vi "Battery Health Checker.vi"(11 "error in":errorcluster) -> (15 "error out":errorcluster)   [LabVIEW 2026]
doc: "Top-level UI of the AA battery health checker. Opens the NI-DMM named in DMM Resource and polls Read Battery Voltage every 200 ms. A battery is detected when |V| >= 0.20 V on 3 consecutive polls; then Measure Battery and Classify Battery run once, the result is shown and a row (time, chemistry, charge, OCV, internal resistance, description) is appended to History. After |V| < 0.10 V on 3 consecutive polls the result is cleared and the VI waits for the next battery. Stop or an error ends the loop; the DMM session is then closed and error out carries the error of the run and of the close."
panel:
  in  "Stop":bool
  out "History":string[][](table)
  out "Measurement":T1
  out "Description":string
  out "Charge (%)":dbl
  out "Chemistry":T2(ring)
  out "Status":string
  out "Battery Present":bool
  out "Live Voltage (V)":dbl
  in  "DMM Resource":refnum<k15>="PXI1Slot3"
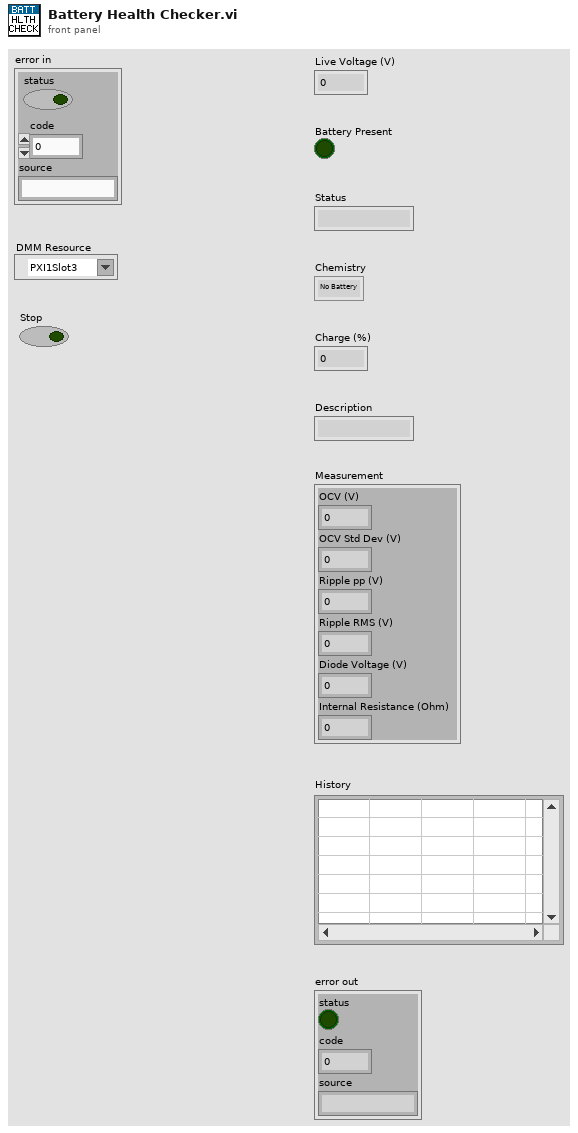
[diagram p1: front panel]
types:
  T1 = cluster{"OCV (V)":dbl, "OCV Std Dev (V)":dbl, "Ripple pp (V)":dbl, "Ripple RMS (V)":dbl, "Diode Voltage (V)":dbl, "Internal Resistance (Ohm)":dbl}
  T2 = enum16{"No Battery", "Reversed Polarity", "Alkaline", "Ni-MH", "Alkaline or Ni-MH", "Li-ion 1.5V (BMS)", "Depleted", "Unknown"}
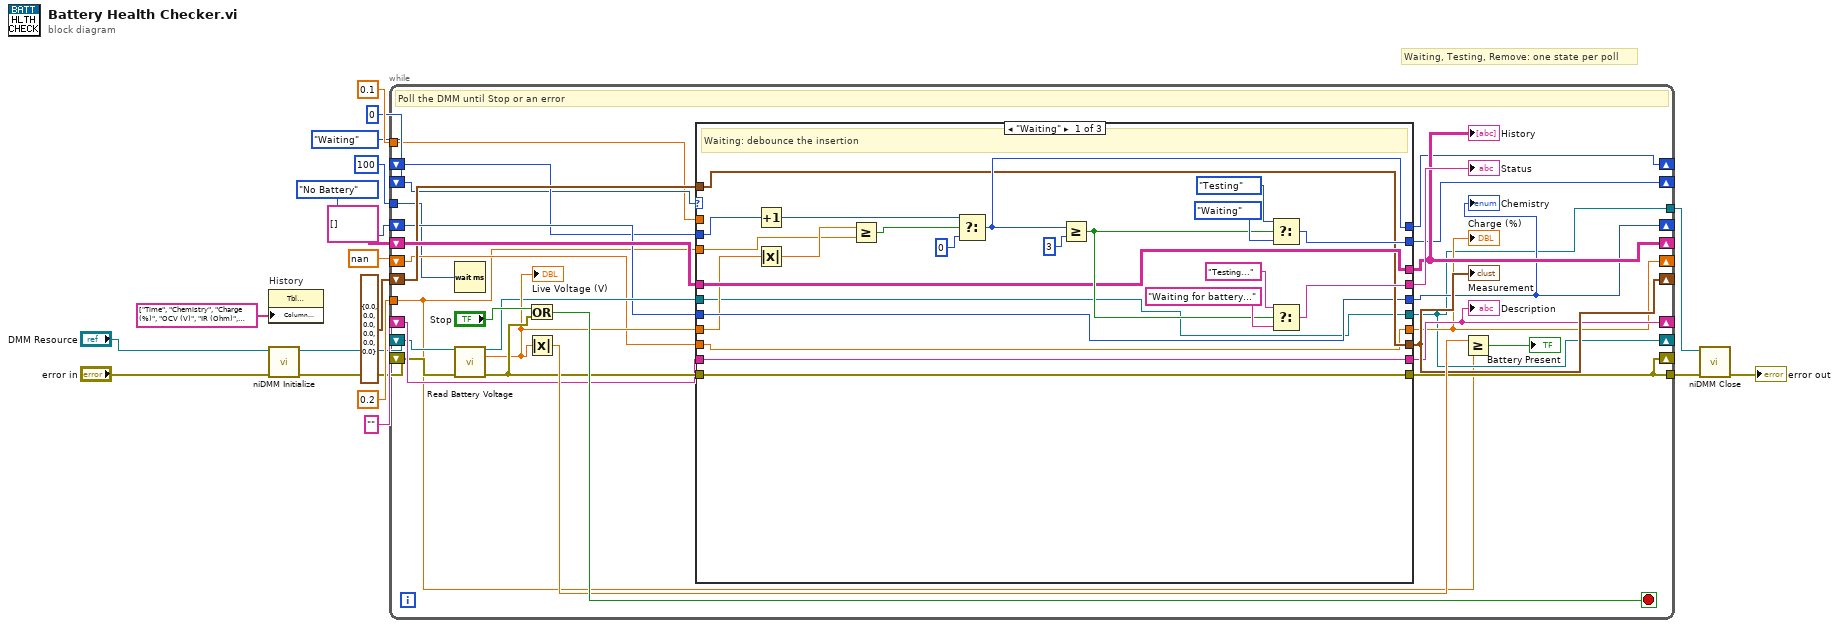
[diagram p0: block diagram]
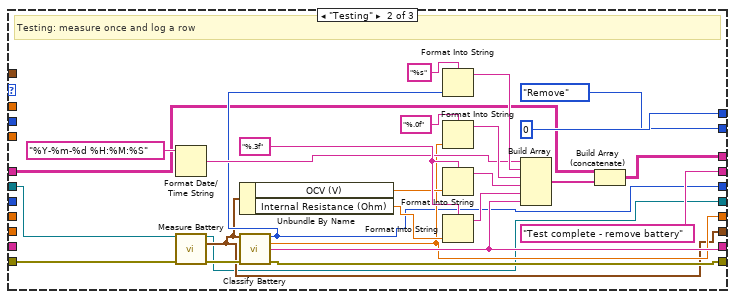
[diagram p2: hidden frame]
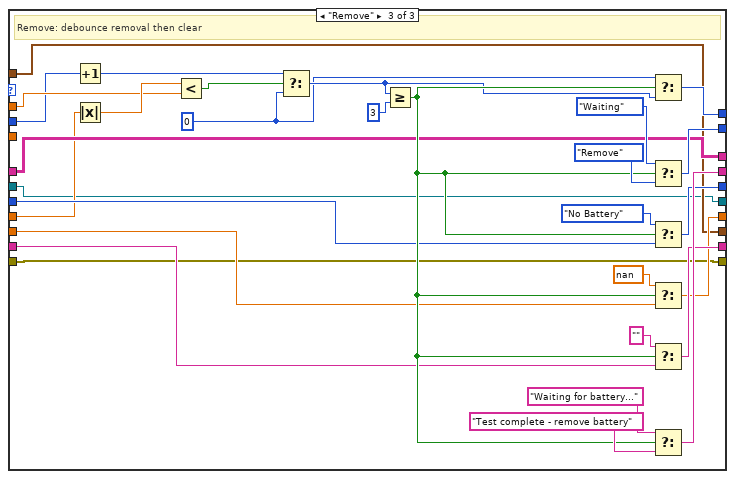
[diagram p3: hidden frame]
diagram:
  # "Waiting, Testing, Remove: one state per poll"
  n1 = property on="History" class="Tbl (strict)"("Column Header Strings[]"=string[] ["Time", "Chemistry", "Charge (%)", "OCV (V)", "IR (Ohm)", "Description"]) -> ()  [unwired: 2 in, 2 out]
  n2 = call <instrlib>:"niDMM Initialize.vi"("error in (no error)"="error in", "Instrument Descriptor"="DMM Resource") -> ("error out"=w4:errorcluster, "instrument handle out"=w5:refnum<k15>)  [unwired: 8 in]
  n3 = while {
    tunnel: 100 ("milliseconds to wait") -> [w19]
    tunnel: 0.2 ("present threshold") -> [w20]
    tunnel: 0.1 ("removed threshold") -> [w21]
    shift-right: [w27] -> _
    shift-left: enum16{"Waiting", "Testing", "Remove"}."Waiting" ("initial state") -> [w26]
    shift-right: [w29] -> _
    shift-left: 0 ("initial count") -> [w28]
    shift-right: [w31] -> _
    shift-left: T2."No Battery" ("initial Chemistry") -> [w30]
    shift-right: [w33] -> _
    shift-left: nan ("initial Charge") -> [w32]
    shift-right: [w35] -> _
    shift-left: "" ("initial Description") -> [w34]
    shift-right: [w37] -> _
    shift-left: T1 {"OCV (V)"=0.0, "OCV Std Dev (V)"=0.0, "Ripple pp (V)"=0.0, "Ripple RMS (V)"=0.0, "Diode Voltage (V)"=0.0, "Internal Resistance (Ohm)"=0.0} ("initial Measurement") -> [w36]
    shift-right: [w39] -> _
    shift-left: string[][] [] ("initial History") -> [w38]
    shift-right: [w23] -> _
    shift-left: w5 -> [w22]
    shift-right: [w25] -> _
    shift-left: w4 -> [w24]
    tunnel: [w23] -> w16
    tunnel: [w25] -> w17
    stop <- w47 stop-if-true
    # "Poll the DMM until Stop or an error"
    n4 = Wait (ms)(milliseconds to wait=w19) -> ()  [unwired: 1 out]
    n5 = call "Read Battery Voltage.vi"("instrument handle"=w22, "error in"=w24) -> ("instrument handle out"=w40:refnum<k15>, "Voltage (V)"=w41:dbl, "error out"=w42:errorcluster)  [unwired: 11 in]
    "Live Voltage (V)" <- w41
    n6 = Or(x="Stop", y=w42) -> (x .or. y?=w47:bool)
    n7 = Absolute Value(x=w41) -> (abs(x)=w43:dbl)
    n8 = case shown="\"Waiting\"" w26 {
      tunnel: w28 -> [w50 _ w99]
      tunnel: w20 -> [w52 _ _]
      tunnel: w30 -> [w53 _ w101]
      tunnel: w32 -> [w54 _ w102]
      tunnel: w34 -> [w55 _ w103]
      tunnel: w36 -> [w56 _ w104]
      tunnel: w38 -> [w57 w73 w105]
      tunnel: w21 -> [_ _ w106]
      tunnel: [w53 w77 w119] -> w31
      tunnel: [w54 w78 w121] -> w33
      tunnel: [w55 w79 w123] -> w35
      tunnel: [w56 w75 w104] -> w37
      tunnel: [w57 w93 w105] -> w39
      tunnel: w40 -> [w48 w71 w97]
      tunnel: w42 -> [w49 w72 w98]
      tunnel: w41 -> [w51 _ w100]
      tunnel: [w48 w74 w97] -> w23
      tunnel: [w49 w80 w98] -> w25
      tunnel: [w62 0 ("count") w114] -> w29
      tunnel: [w67 enum16{"Waiting", "Testing", "Remove"}."Remove" ("next state") w117] -> w27
      tunnel: [w70 "Test complete - remove battery" ("Status") w126] -> w45
      frame "Waiting" {
        # "Waiting: debounce the insertion"
        n9 = Increment(x=w50) -> (x+1=w60:i32)
        n10 = Absolute Value(x=w51) -> (abs(x)=w58:dbl)
        n11 = Greater Or Equal?(x=w58, y=w52) -> (x >= y?=w59:bool)
        n12 = Select(t=w60, s=w59, f=0) -> (s? t:f=w62:i32)
        n13 = Greater Or Equal?(x=w62, y=3) -> (x >= y?=w64:bool)
        n14 = Select(t=enum16{"Waiting", "Testing", "Remove"}."Testing", s=w64, f=enum16{"Waiting", "Testing", "Remove"}."Waiting") -> (s? t:f=w67:enum16{"Waiting", "Testing", "Remove"})
        n15 = Select(t="Testing...", s=w64, f="Waiting for battery...") -> (s? t:f=w70:string)
      }
      frame "Testing" {
        w89 = "%.3f" ("format string")
        # "Testing: measure once and log a row"
        n16 = Format Date/Time String(time format string (%c)="%Y-%m-%d %H:%M:%S") -> (date/time string=w82:string)  [unwired: 1 in, 1 out]
        n17 = call "Measure Battery.vi"("instrument handle"=w71, "error in"=w72) -> ("instrument handle out"=w74:refnum<k15>, "Measurement"=w75:T1, "error out"=w76:errorcluster)  [unwired: 11 in]
        n18 = Unbundle By Name(w75) -> ("OCV (V)"=w87:dbl, "Internal Resistance (Ohm)"=w88:dbl)
        n19 = call "Classify Battery.vi"("Measurement"=w75, "error in"=w76) -> ("Chemistry"=w77:T2, "Charge (%)"=w78:dbl, "Description"=w79:string, "error out"=w80:errorcluster)  [unwired: 10 in]
        n20 = Format Into String(format string="%s", w77) -> (resulting string=w84:string)  [unwired: 2 in, 1 out]
        n21 = Format Into String(format string="%.0f", w78) -> (resulting string=w86:string)  [unwired: 2 in, 1 out]
        n22 = Format Into String(format string=w89, w87) -> (resulting string=w90:string)  [unwired: 2 in, 1 out]
        n23 = Format Into String(format string=w89, w88) -> (resulting string=w91:string)  [unwired: 2 in, 1 out]
        n24 = Build Array(w82, w84, w86, w90, w91, w79) -> (w92:string[])
        n25 = Build Array (concatenate)(w73, w92) -> (w93:string[][])
      }
      frame "Remove" {
        w110 = 0 ("f")
        # "Remove: debounce removal then clear"
        n26 = Increment(x=w99) -> (x+1=w109:i32)
        n27 = Absolute Value(x=w100) -> (abs(x)=w107:dbl)
        n28 = Less?(x=w107, y=w106) -> (x < y?=w108:bool)
        n29 = Select(t=w109, s=w108, f=w110) -> (s? t:f=w111:i32)
        n30 = Greater Or Equal?(x=w111, y=3) -> (x >= y?=w113:bool)
        n31 = Select(t=w110, s=w113, f=w111) -> (s? t:f=w114:i32)
        n32 = Select(t=enum16{"Waiting", "Testing", "Remove"}."Waiting", s=w113, f=enum16{"Waiting", "Testing", "Remove"}."Remove") -> (s? t:f=w117:enum16{"Waiting", "Testing", "Remove"})
        n33 = Select(t=T2."No Battery", s=w113, f=w101) -> (s? t:f=w119:T2)
        n34 = Select(t=nan, s=w113, f=w102) -> (s? t:f=w121:dbl)
        n35 = Select(t="", s=w113, f=w103) -> (s? t:f=w123:string)
        n36 = Select(t="Waiting for battery...", s=w113, f="Test complete - remove battery") -> (s? t:f=w126:string)
      }
    }
    "Status" <- w45
    "Chemistry" <- w31
    "Charge (%)" <- w33
    "Description" <- w35
    "Measurement" <- w37
    "History" <- w39
    n37 = Greater Or Equal?(x=w43, y=w20) -> (x >= y?=→"Battery Present":bool)
  }
  n38 = call <instrlib>:"niDMM Close.vi"("error in (no error)"=w17, "instrument handle"=w16) -> ("error out"=→"error out":errorcluster)  [unwired: 9 in]
